vi "InitialConditionTest.vi"(0 "VI Reference In":refnum<vi>, 11 "error in":errorcluster) -> (4 "VI Reference Out":refnum<vi>, 15 "error out":errorcluster)   [LabVIEW 2016, in "CarWashTest.lvlib"]
doc: "Initial condition test"
uses:
  CarWashTest.lvlib
  Solution/Controls/Wash Options.ctl
  Solution/Controls/Car Wash Indicators.ctl
  APIs/Assert/AssertControlProperty/AssertControlDisable/AssertEnabled.vi
  APIs/Assert/AssertControlValue/Equal.vi
  <vilib>/addons/_JKI Toolkits/Caraya/classes/Test/Test.lvclass
  Drona.lvlib
  APIs/Assert/AssertControlValue/AssertControlValue.lvlib
  APIs/Assert/AssertControlProperty/AssertControlDisable/AssertControlDisable.lvlib
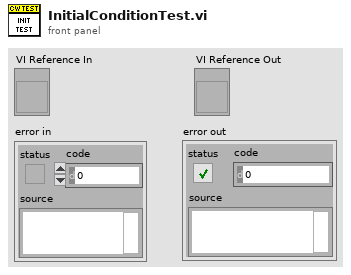
[diagram p1: front panel]
types:
  T1 = typedef "Car Wash Indicators.ctl" = cluster{"Under Body Wash":bool, "Bug Remover":bool, "Pre-Soak":bool, "High Pressure Wash":bool, "Low Pressure Wax":bool, "Spot Free Rinse":bool, "Tire Shine Foam":bool, "Air Dry":bool, "Vehicle Out of Position":bool}
  T2 = typedef "Wash Options.ctl" = cluster{"Under Body Wash":bool, "Bug Remover":bool, "Pre-Soak":bool, "High Pressure Wash":bool, "Low Pressure Wax":bool, "Spot Free Rinse":bool, "Tire Shine Foam":bool, "Air Dry":bool}
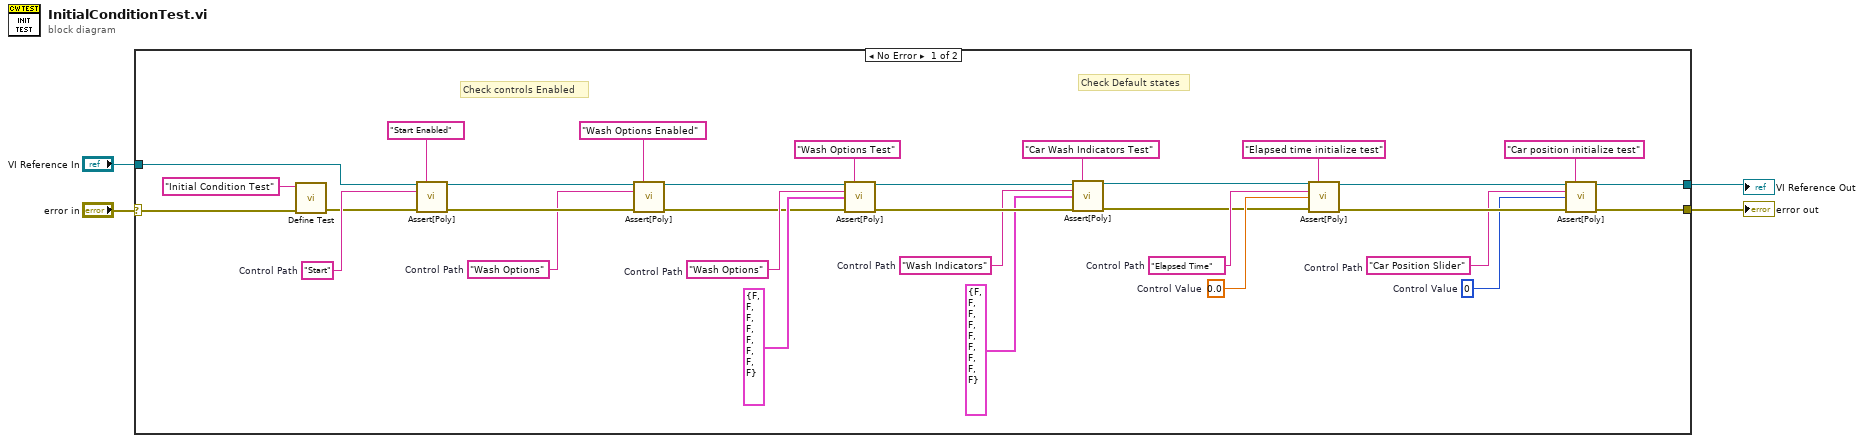
[diagram p0: block diagram]
diagram:
  n1 = case shown="No Error" "error in" {
    selector: "error in" -> [w16 w37]
    tunnel: [w18 w37] -> w4
    tunnel: [w17 w38] -> w3
    tunnel: "VI Reference In" -> [w6 w38]
    frame No Error {
      w11 = "Start"  # Control Path
      w9 = "Wash Options"  # Control Path
      w21 = "Wash Indicators"  # Control Path
      w28 = "Wash Options"  # Control Path
      w29 = 0  # Control Value
      w30 = "Car Position Slider"  # Control Path
      w35 = 0.0  # Control Value
      w36 = "Elapsed Time"  # Control Path
      # "Check Default states"
      # "Check controls Enabled"
      n2 = call <vilib>:"Define Test.vi"("error in (no error)"=w16, "Label (VI Title)"="Initial Condition Test") -> ("error out"=w8:errorcluster)  [unwired: 8 in, 1 out]
      n3 = call-poly "Assert[Poly].vi"("VI Reference In"=w6, "Test Label"="Start Enabled", "Control Path"=w11, "Error In"=w8) -> ("VI Reference Out"=w13:refnum<vi>, "Error Out"=w12:errorcluster)  [unwired: 9 in, 1 out]
      n4 = call-poly "Assert[Poly].vi"("VI Reference In"=w13, "Test Label"="Wash Options Enabled", "Control Path"=w9, "Error In"=w12) -> ("VI Reference Out"=w5:refnum<vi>, "Error Out"=w7:errorcluster)  [unwired: 9 in, 1 out]
      n5 = call-poly "Assert[Poly].vi"("VI Reference In"=w5, "Test Label"="Wash Options Test", "Control Path"=w28, "Control Value"=T2 {"Under Body Wash"=FALSE, "Bug Remover"=FALSE, "Pre-Soak"=FALSE, "High Pressure Wash"=FALSE, "Low Pressure Wax"=FALSE, "Spot Free Rinse"=FALSE, "Tire Shine Foam"=FALSE, "Air Dry"=FALSE} ("Wash Options"), "Error In"=w7) -> ("VI Reference Out"=w22:refnum<vi>, "Error Out"=w25:errorcluster)  [unwired: 8 in, 1 out]
      n6 = call-poly "Assert[Poly].vi"("VI Reference In"=w22, "Test Label"="Car Wash Indicators Test", "Control Path"=w21, "Control Value"=T1 {"Under Body Wash"=FALSE, "Bug Remover"=FALSE, "Pre-Soak"=FALSE, "High Pressure Wash"=FALSE, "Low Pressure Wax"=FALSE, "Spot Free Rinse"=FALSE, "Tire Shine Foam"=FALSE, "Air Dry"=FALSE, "Vehicle Out of Position"=FALSE} ("Car Wash Indicators"), "Error In"=w25) -> ("VI Reference Out"=w23:refnum<vi>, "Error Out"=w24:errorcluster)  [unwired: 8 in, 1 out]
      n7 = call-poly "Assert[Poly].vi"("VI Reference In"=w23, "Test Label"="Elapsed time initialize test" ("Label"), "Control Path"=w36, "Control Value"=w35, "Error In"=w24) -> ("VI Reference Out"=w31:refnum<vi>, "Error Out"=w32:errorcluster)  [unwired: 8 in, 1 out]
      n8 = call-poly "Assert[Poly].vi"("VI Reference In"=w31, "Test Label"="Car position initialize test" ("Label"), "Control Path"=w30, "Control Value"=w29, "Error In"=w32) -> ("VI Reference Out"=w17:refnum<vi>, "Error Out"=w18:errorcluster)  [unwired: 8 in, 1 out]
    }
    frame Error {
    }
  }
  "error out" <- w4
  "VI Reference Out" <- w3
